vi "Init Node.vi"(7 "First Launch":bool, 8 "error in (no error)":errorcluster, 11 "Volatus Core in":refnum<class "Volatus Core.lvclass">) -> (0 "error out":errorcluster, 3 "Volatus Core out":refnum<class "Volatus Core.lvclass">)   [LabVIEW 2020, in "Volatus.lvlib" / "Volatus Core.lvclass"]
uses:
  Volatus Core.lvclass
  C:/dev/lv20CE/relink/lv-volatus/Volatus/Module/Module.lvclass
  Event Reporter Module/Event Reporter Module.lvclass
  Module/Module.lvclass
  Module/Module.lvclass/Module.ctl
  Volatus Core.lvclass/Volatus Core.ctl
  MessageQ/MessageQ.lvclass/MessageQ.ctl
  MessageQ/Send.vi
  VolatusAPI/VolatusAPI.lvclass
  C:/dev/lv20CE/relink/lv-volatus/Volatus/Volatus Core/Volatus Core.lvclass
  C:/dev/lv20CE/relink/lv-volatus/Volatus/Event Reporter Module/Event Reporter Module.lvclass
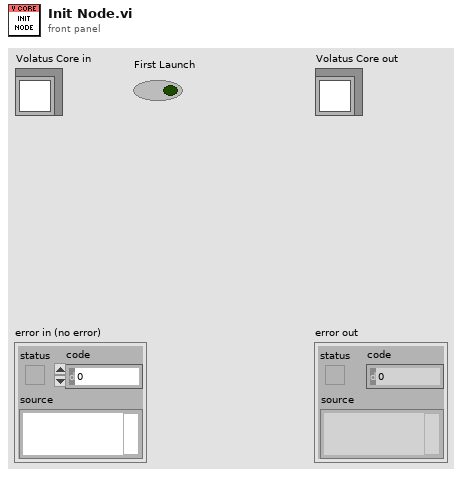
[diagram p1: front panel]
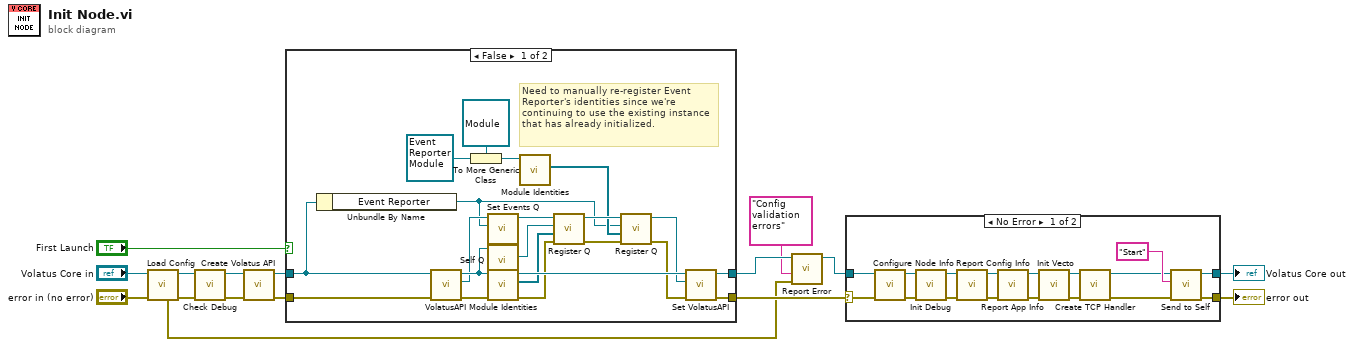
[diagram p0: block diagram]
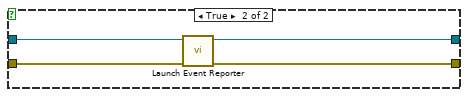
[diagram p2: hidden frame]
diagram:
  n1 = call "Load Config.vi"("error in (no error)"="error in (no error)", "Volatus Core in"="Volatus Core in") -> ("error out"=w16:errorcluster, "Volatus Core out"=w8:refnum<class "Volatus Core.lvclass">, "Validation Errors"=w2:errorcluster)  [unwired: 7 in]
  n2 = call "Check Debug.vi"("error in (no error)"=w16, "Volatus Core in"=w8) -> ("error out"=w9:errorcluster, "Volatus Core out"=w7:refnum<class "Volatus Core.lvclass">)  [unwired: 8 in]
  n3 = call "Create Volatus API.vi"("error in (no error)"=w9, "Volatus Core in"=w7) -> ("error out"=w12:errorcluster, "Volatus Core out"=w11:refnum<class "Volatus Core.lvclass">)  [unwired: 8 in]
  n4 = case shown="False" "First Launch" {
    tunnel: w12 -> [w26 w39]
    tunnel: w11 -> [w27 w37]
    tunnel: [w18 w38] -> w3
    tunnel: [w28 w36] -> w5
    frame False {
      # "Need to manually re-register Event Reporter's identities since we're continuing to use the existing instance that has already initialized."
      n5 = Unbundle By Name(w27) -> ("Event Reporter"=w22:refnum<class "MessageQ.lvclass">)
      n6 = call "VolatusAPI.vi"("Module in"=w27) -> ("VolatusAPI"=w29:refnum<class "VolatusAPI.lvclass">, "Module out"=w32:refnum<class "Volatus Core.lvclass">)  [unwired: 9 in]
      n7 = To More Generic Class(target class=refnum<class "Module.lvclass"> refnum ("Volatus:Module"), reference=refnum<class "Event Reporter Module.lvclass"> refnum ("Event Reporter Module in")) -> (generic class reference=w20:refnum<class "Module.lvclass">)
      n8 = call "Set Events Q.vi"("Events Q"=w22, "VolatusAPI in"=w29) -> ("VolatusAPI out"=w30:refnum<class "VolatusAPI.lvclass">)  [unwired: 9 in]
      n9 = call "Self Q.vi"("Module in"=w32) -> ("Self Q"=w33:refnum<class "MessageQ.lvclass">)  [unwired: 9 in, 1 out]
      n10 = call-dynamic "Module Identities.vi"("error in (no error)"=w26, "Volatus Core in"=w32) -> ("error out"=w34:errorcluster, "Identities"=w31:refnum<class "Identity.lvclass">[], "Volatus Core out"=w35:refnum<class "Volatus Core.lvclass">)  [unwired: 7 in]
      n11 = call-dynamic "Module Identities.vi"("Module in"=w20) -> ("Identities"=w23:refnum<class "Identity.lvclass">[])  [unwired: 8 in, 2 out]
      n12 = call "Register Q.vi"("error in (no error)"=w34, "Identities"=w31, "MessageQ"=w33, "VolatusAPI in"=w30) -> ("error out"=w24:errorcluster, "VolatusAPI out"=w25:refnum<class "VolatusAPI.lvclass">)  [unwired: 5 in, 1 out]
      n13 = call "Register Q.vi"("error in (no error)"=w24, "Identities"=w23, "MessageQ"=w22, "VolatusAPI in"=w25) -> ("error out"=w18:errorcluster, "VolatusAPI out"=w17:refnum<class "VolatusAPI.lvclass">)  [unwired: 5 in, 1 out]
      n14 = call "Set VolatusAPI.vi"("VolatusAPI"=w17, "Module in"=w35) -> ("Module out"=w28:refnum<class "Volatus Core.lvclass">)  [unwired: 9 in]
    }
    frame True {
      n15 = call "Launch Event Reporter.vi"("error in (no error)"=w39, "Volatus Core in"=w37) -> ("error out"=w38:errorcluster, "Volatus Core out"=w36:refnum<class "Volatus Core.lvclass">)  [unwired: 8 in]
    }
  }
  n16 = call "Report Error.vi"("error in (no error)"=w2, "Message (None)"="Config validation errors", "Module in"=w5) -> ("Module out"=w4:refnum<class "Volatus Core.lvclass">)  [unwired: 7 in, 1 out]
  n17 = case shown="No Error" w3 {
    selector: w3 -> [w56 w57]
    tunnel: w4 -> [w47 w58]
    tunnel: [w51 w58] -> w14
    tunnel: [w52 w57] -> w13
    frame No Error {
      n18 = call "Configure Node Info.vi"("error in (no error)"=w56, "Volatus Core in"=w47) -> ("error out"=w48:errorcluster, "Volatus Core out"=w43:refnum<class "Volatus Core.lvclass">)  [unwired: 8 in]
      n19 = call "Init Debug.vi"("error in (no error)"=w48, "Volatus Core in"=w43) -> ("error out"=w44:errorcluster, "Volatus Core out"=w42:refnum<class "Volatus Core.lvclass">)  [unwired: 8 in]
      n20 = call "Report Config Info.vi"("error in (no error)"=w44, "Volatus Core in"=w42) -> ("error out"=w46:errorcluster, "Volatus Core out"=w45:refnum<class "Volatus Core.lvclass">)  [unwired: 8 in]
      n21 = call "Report App Info.vi"("error in (no error)"=w46, "Volatus Core in"=w45) -> ("error out"=w55:errorcluster, "Volatus Core out"=w53:refnum<class "Volatus Core.lvclass">)  [unwired: 8 in]
      n22 = call "Init Vecto.vi"("error in (no error)"=w55, "Volatus Core in"=w53) -> ("error out"=w54:errorcluster, "Volatus Core out"=w49:refnum<class "Volatus Core.lvclass">)  [unwired: 8 in]
      n23 = call "Create TCP Handler.vi"("error in (no error)"=w54, "Volatus Core in"=w49) -> ("error out"=w40:errorcluster, "Volatus Core out"=w41:refnum<class "Volatus Core.lvclass">)  [unwired: 8 in]
      n24 = call "Send to Self.vi"("error in (no error)"=w40, "Message ID"="Start", "Module in"=w41) -> ("error out"=w52:errorcluster, "Module out"=w51:refnum<class "Volatus Core.lvclass">)  [unwired: 7 in]
    }
    frame Error {
    }
  }
  "error out" <- w13
  "Volatus Core out" <- w14
